vi "Read Generated files.vi"(11 "BuildManager in":refnum<class "BuildManager.lvclass">) -> (2 "Generated file":T1, 3 "BuildManager out":refnum<class "BuildManager.lvclass">)   [LabVIEW 2019, in "SolutionBuilder.lvlib" / "BuildManager.lvclass"]
uses:
  BuildManager.lvclass
  GeneratedFile.ctl
  BuildManager.lvclass/BuildManager.ctl
  BuildProjectInfo.ctl
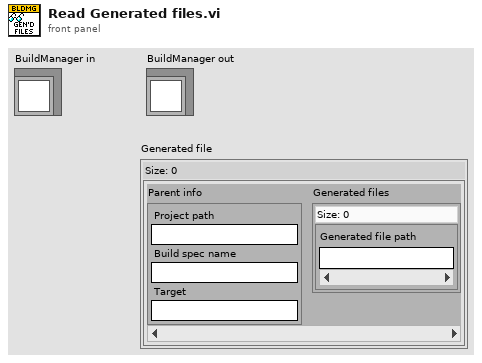
[diagram p1: front panel]
types:
  T1 = typedef "SolutionBuilder.lvlib/BuildManager.lvclass/GeneratedFile.ctl" = map{T2, set{string}}
  T2 = typedef "SolutionBuilder.lvlib/BuildManager.lvclass/BuildProjectInfo.ctl" = cluster{"Project path":string, "Build spec name":string, "Target":string}
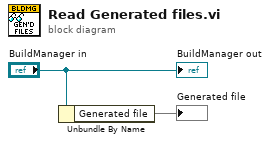
[diagram p0: block diagram]
diagram:
  n1 = Unbundle By Name("BuildManager in") -> ("Generated file"=→"Generated file":T1)
  "BuildManager out" <- "BuildManager in"
